vi "Display Message Dialog.vi"(8 "error in":errorcluster, 11 "Message to display":string) -> (0 "error out":errorcluster)   [LabVIEW 2020, in "SEECD System Explorer.lvlib"]
uses:
  SEECD System Explorer.lvlib
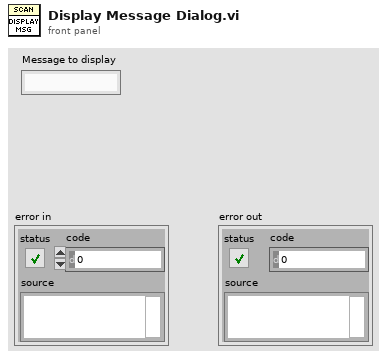
[diagram p1: front panel]
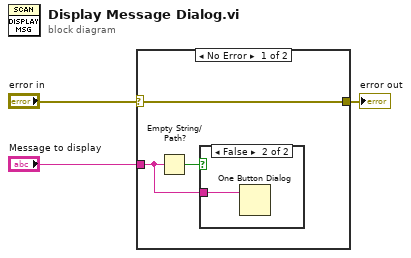
[diagram p0: block diagram]
diagram:
  n1 = case shown="No Error" "error in" {
    selector: "error in" -> [w6 w8]
    tunnel: [w6 w8] -> w2
    tunnel: "Message to display" -> [w4 _]
    frame No Error {
      n2 = Empty String/Path?(string/path=w4) -> (empty?=w5:bool)
      n3 = case shown="False" w5 {
        tunnel: w4 -> [_ w7]
        frame True {
        }
        frame False {
          n4 = One Button Dialog(message=w7) -> ()  [unwired: 1 in, 1 out]
        }
      }
    }
    frame Error {
    }
  }
  "error out" <- w2
